vi "GT_AlarmText.vi"(11 "Alarm Code":u16) -> (3 "Alarm Text":string)   [LabVIEW 2026]
doc: "Use this template to build a VI to use as a subVI."
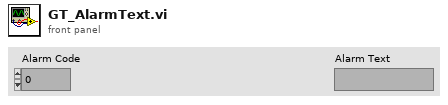
[diagram p1: front panel]
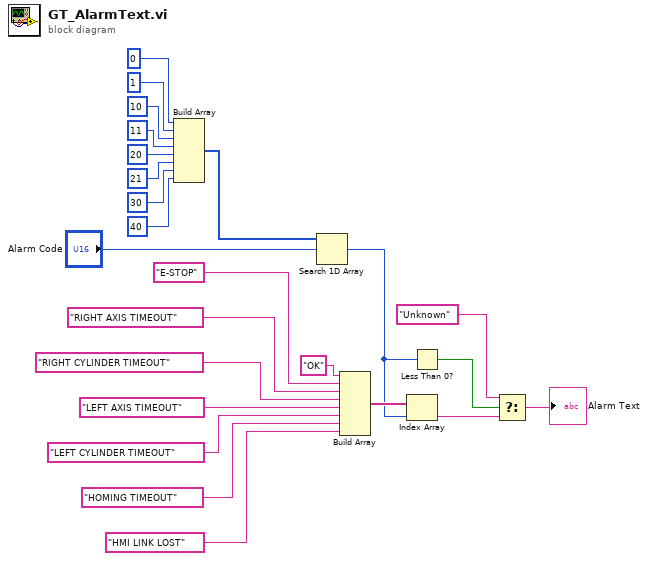
[diagram p0: block diagram]
diagram:
  n1 = Build Array(0, 1, 10, 11, 20, 21, 30, 40) -> (w8:i32[])
  n2 = Search 1D Array(1D array=w8, element="Alarm Code") -> (index of element=w5:i32)  [unwired: 1 in]
  n3 = Build Array("OK", "E-STOP", "RIGHT AXIS TIMEOUT", "RIGHT CYLINDER TIMEOUT", "LEFT AXIS TIMEOUT", "LEFT CYLINDER TIMEOUT", "HOMING TIMEOUT", "HMI LINK LOST") -> (w6:string[])
  n4 = Index Array(array=w6, index=w5) -> (element=w2:string)
  n5 = Less Than 0?(x=w5) -> (x < 0?=w4:bool)
  n6 = Select(t="Unknown", s=w4, f=w2) -> (s? t:f=→"Alarm Text":string)
